vi "lvssh2_userauth_keyboard_interactive_response_function_handler_64.vi"(9 "lvssh2_userauth_keyboard_interactive_response_function":refnum<vi>, 10 "Stop Event Ref":refnum<user-event>, 11 "User Event Ref":refnum<user-event>) -> ()   [LabVIEW 2017, in "libssh2.lvlib"]
uses:
  libssh2.lvlib
  lvssh2_userauth_keyboard_interactive_response_function_input_args_64.ctl
  lvssh2_userauth_keyboard_interactive_prompt.ctl
  lvssh2_extensions_64.dll
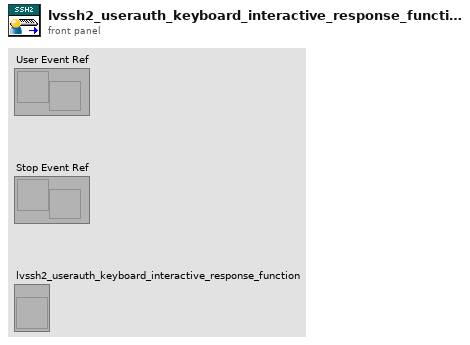
[diagram p1: front panel]
types:
  T1 = typedef "libssh2.lvlib/lvssh2_userauth_keyboard_interactive_prompt.ctl" = cluster{"text":string, "echo":bool}
  T2 = cluster{"text":u64, "length":u64, "echo":u8, "padding-1":u8, "padding-2":u16, "padding-3":u32}
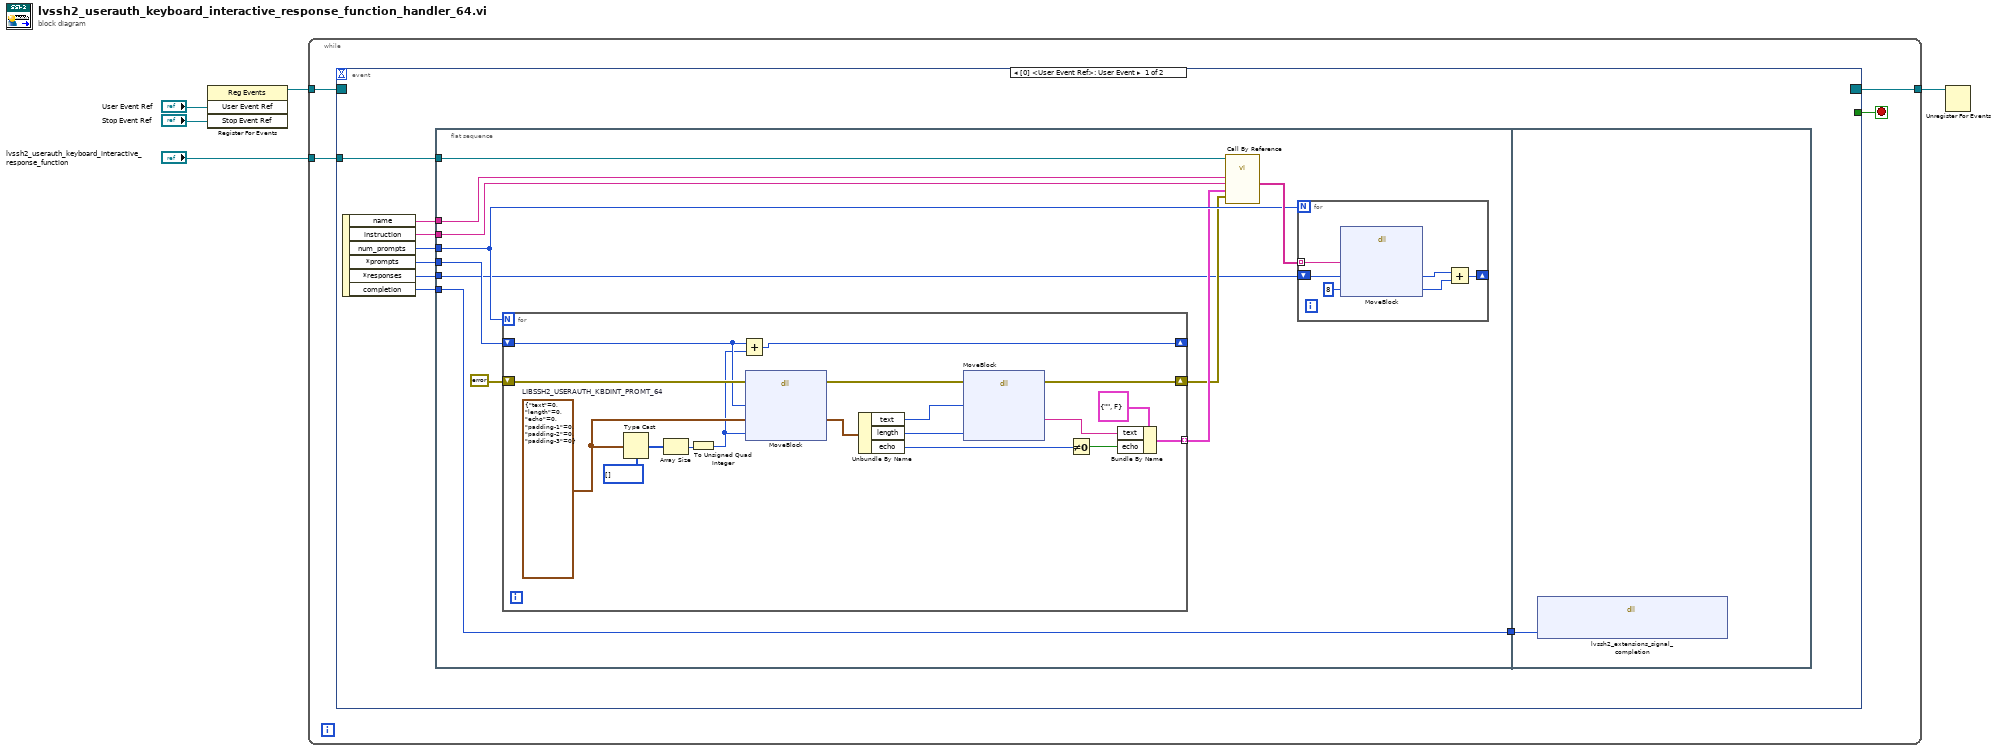
[diagram p0: block diagram]
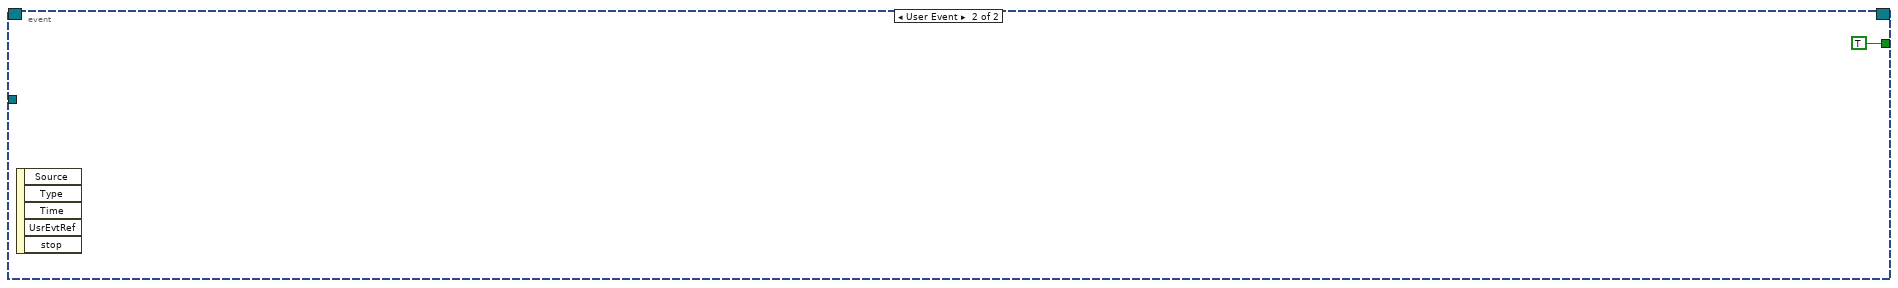
[diagram p2: hidden frame]
diagram:
  n1 = register-events("User Event Ref", "Stop Event Ref") -> (reference out=w2:refnum<event-registration>)  [unwired: 2 in, 1 out]
  n2 = while {
    tunnel: "lvssh2_userauth_keyboard_interactive_response_function" -> [w9]
    tunnel: [w8] -> w4
    tunnel: w2 -> [w7]
    stop <- w6 stop-if-true
    n3 = event shown="[0] <User Event Ref>: User Event" {
      selector: w7 -> [_ _]
      dyn-events: [_ _] -> w8
      timeout: _ -> [_ _]
      tunnel: w9 -> [w16 _]
      tunnel: [_ TRUE] -> w6
      event User Event {
        n4 = event-data() -> ("name"=w15:string, "instruction"=w14:string, "num_prompts"=w13:i32, "*prompts"=w12:u64, "*responses"=w11:u64, "completion"=w10:u64)  [unwired: 1 in]
        n5 = flat-sequence {
          tunnel: w16 -> [w28]
          tunnel: w15 -> [w27]
          tunnel: w14 -> [w26]
          tunnel: w13 -> [w24]
          tunnel: w12 -> [w23]
          tunnel: w11 -> [w19]
          tunnel: [w18] -> w17
          tunnel: w10 -> [w18]
          tunnel: w17 -> [w53]
          frame #0 {
            n6 = for {
              N: w24 -> [_]
              tunnel: [w43] -> w22 mode=indexing
              shift-right: [w42] -> _
              shift-left: w23 -> [w39]
              shift-right: [w41] -> w21
              shift-left: errorcluster {"status"=FALSE, "code"=0, "source"=""} ("error out") -> [w40]
              w52 = T2 {"text"=0, "length"=0, "echo"=0, "padding-1"=0, "padding-2"=0, "padding-3"=0}  # LIBSSH2_USERAUTH_KBDINT_PROMT_64
              n7 = Type Cast(type=u8[] [], x=w52) -> (*(type *) &x=w50:u8[])
              n8 = Array Size(array=w50) -> (size(s)=w38:i32)
              n9 = To Unsigned Quad Integer(1:w38) -> (0:w37:u64)
              n10 = Add(x=w39, y=w37) -> (x+y=w42:u64)
              n11 = dll-call lib="LabVIEW" fn="MoveBlock"(error in=w40, "ps"=w39, "pd"=w52, "size"=w37) -> (error out=w49:errorcluster, "pd"=w48:T2)  [unwired: 5 in, 1 out]
              n12 = Unbundle By Name(w48) -> ("text"=w47:u64, "length"=w36:u64, "echo"=w45:u8)
              n13 = dll-call lib="LabVIEW" fn="MoveBlock"(error in=w49, "ps"=w47, "size"=w36) -> (error out=w41:errorcluster, "pd"=w35:string)  [unwired: 6 in, 1 out]
              n14 = Not Equal To 0?(x=w45) -> (x != 0?=w44:bool)
              n15 = Bundle By Name(cluster=T1 {"text"="", "echo"=FALSE} ("prompt"), "text"=w35, "echo"=w44) -> (w43:T1)
            }
            n16 = call-by-ref "?"(reference=w28, "error in (no error)"=w21, "prompts"=w22, "instruction"=w26, "name"=w27) -> ("responses"=w25:string[])  [unwired: 7 in, 3 out]
            n17 = for {
              N: w24 -> [_]
              tunnel: w25 -> [w32] mode=indexing
              shift-right: [w30] -> _
              shift-left: w19 -> [w33]
              n18 = dll-call lib="LabVIEW" fn="MoveBlock"("ps"=w32, "pd"=w33, "size"=u64 8) -> ("pd"=w31:u64, "size"=w29:u64)  [unwired: 5 in, 2 out]
              n19 = Add(x=w31, y=w29) -> (x+y=w30:u64)
            }
          }
          frame #1 {
            n20 = dll-call lib="C:/Users/Pascal/Projects/Home/lvssh2/libssh2/lvssh2_extensions**.*" fn="lvssh2_extensions_signal_completion"("completion"=w53) -> ()  [unwired: 5 in, 2 out]
          }
        }
      }
      event User Event {
        n21 = event-data() -> ()  [unwired: 1 in, 5 out]
      }
    }
  }
  n22 = Unregister For Events(event registration refnum=w4) -> ()  [unwired: 1 in, 1 out]
